vi "ReadTemplateData.vi"(8 "error in (no error)":errorcluster, 11 "object in":refnum<class "Template_CFG.lvclass">) -> (0 "error out":errorcluster, 2 "Data":T1, 3 "object out":refnum<class "Template_CFG.lvclass">)   [LabVIEW 2021, in "Template-Channels.lvlib" / "Template_CFG.lvclass"]
uses:
  Template_CFG.lvclass
  tdef/Data.ctl
  Template_CFG.lvclass/Template_CFG.ctl
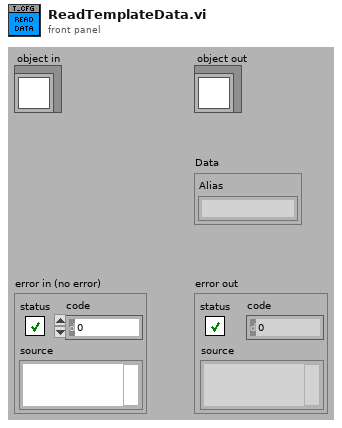
[diagram p1: front panel]
types:
  T1 = typedef "Template-Channels.lvlib/Template_CFG.lvclass/Data.ctl" = cluster{"Alias":string}
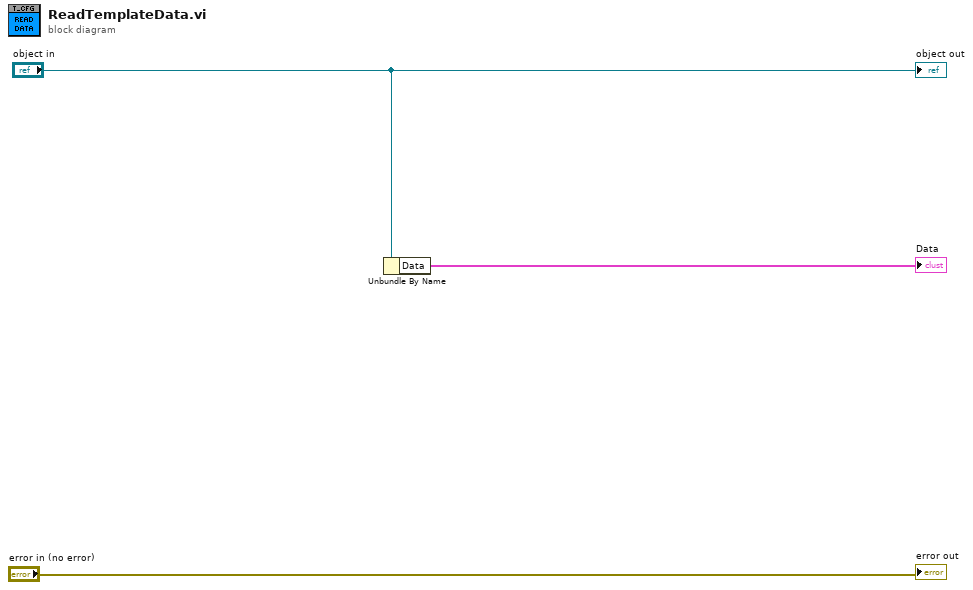
[diagram p0: block diagram]
diagram:
  n1 = Unbundle By Name("object in") -> ("Data"=→"Data":T1)
  "error out" <- "error in (no error)"
  "object out" <- "object in"
